vi "Compare Ports.vi"(9 "refresh listbox":T8[](array[typedef]), 10 "new port":T1, 11 "old port":T1) -> (1 "refresh listbox out":T8[](array[typedef]))   [LabVIEW 2020, in "Ballard ARINC 429 System Explorer.lvlib" / "Implementation.lvlib"]
uses:
  Implementation.lvlib
  Types/Refresh Listbox.ctl
  Types/Refresh Symbols.ctl
  Shared/VS Channels Definition for All Labels on Hardware Channel.ctl
  Shared/Direction.ctl
  Shared/VS Channels Definition for Label.ctl
  Shared/VS Channel Definition for Parameter.ctl
  Shared/Parameter Definition.ctl
  <vilib>/NI/NI VeriStand Encoding and Decoding/Encoding.ctl
  Shared/Transfer Type.ctl
  <vilib>/NI/NI VeriStand Encoding and Decoding/Encoding and Decoding.lvlib
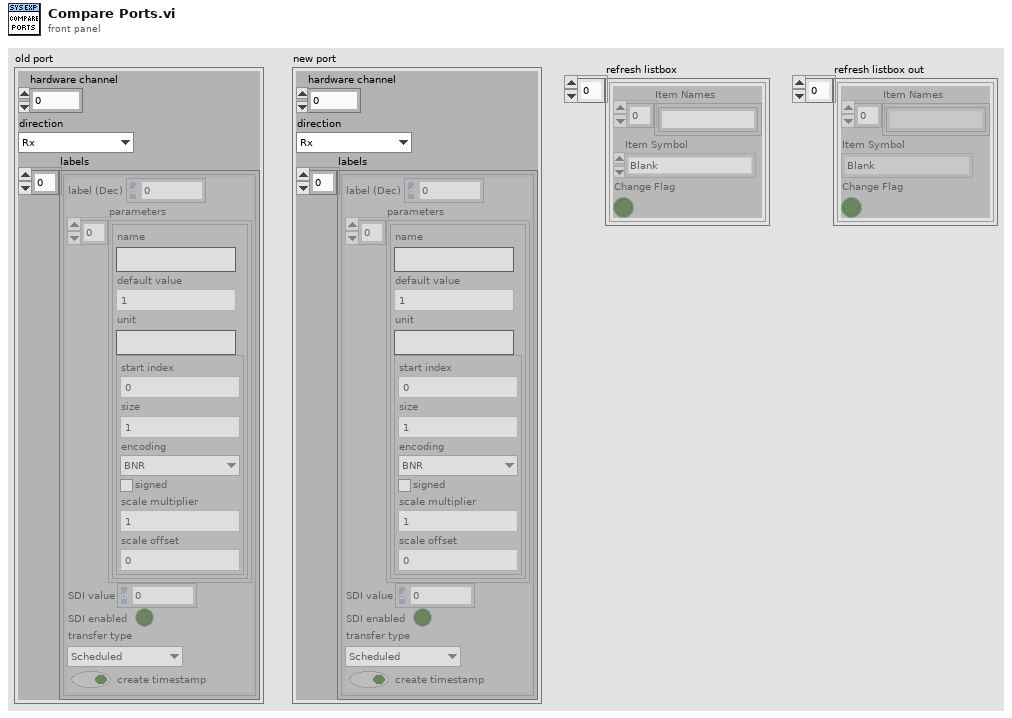
[diagram p1: front panel]
types:
  T1 = typedef "VS Channels Definition for All Labels on Hardware Channel.ctl" = cluster{"hardware channel":i32, "direction":T2, "labels":T3[]}
  T2 = typedef "Direction.ctl" = enum16{"Rx", "Tx"}
  T3 = typedef "VS Channels Definition for Label.ctl" = cluster{"label (Dec)":u32, "parameters":T4[], "SDI value":u8, "SDI enabled":bool, "transfer type":T7, "create timestamp":bool}
  T4 = typedef "VS Channel Definition for Parameter.ctl" = cluster{"name":string, "default value":dbl, "unit":string, "Parameter":T5}
  T5 = typedef "Parameter Definition.ctl" = cluster{"start index":i32, "size":i32, "encoding":T6, "signed":bool, "scale multiplier":dbl, "scale offset":dbl}
  T6 = typedef "Encoding and Decoding.lvlib/Encoding.ctl" = enum16{"BNR", "BCD", "Discrete"}
  T7 = typedef "Transfer Type.ctl" = enum16{"Scheduled", "Acyclic", "Block", "Strobe"}
  T8 = typedef "Ballard ARINC 429 System Explorer.lvlib/Implementation.lvlib/Refresh Listbox.ctl" = cluster{"Item Names":string[], "Item Symbol":T9, "Change Flag":bool}
  T9 = typedef "Ballard ARINC 429 System Explorer.lvlib/Implementation.lvlib/Refresh Symbols.ctl" = enum16{"Blank", "Port", "Incoming", "Outgoing", "Label", "Word", "Parameter", "ARINC-429", "Config Files", "Channel Spec", "Item"}
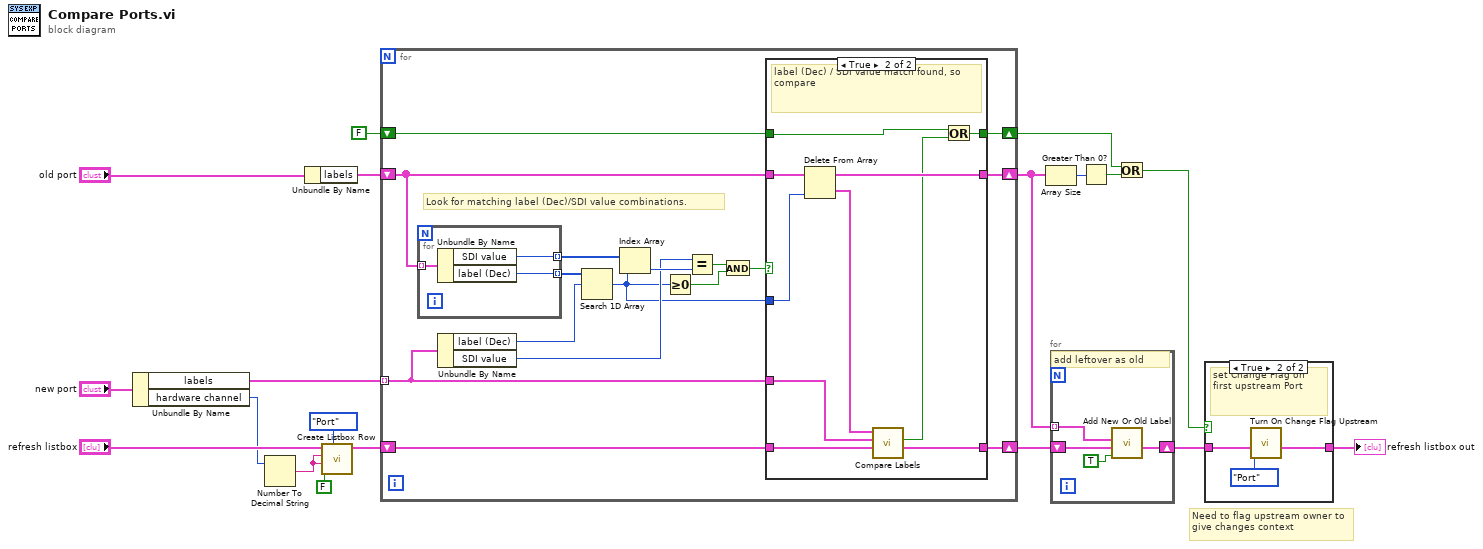
[diagram p0: block diagram]
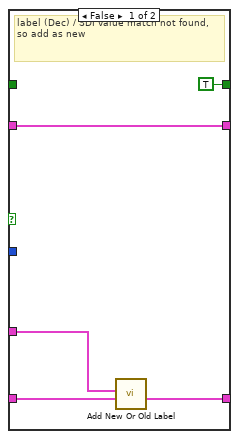
[diagram p3: hidden frame]
diagram:
  # "Need to flag upstream owner to give changes context"
  n1 = Unbundle By Name("new port") -> ("labels"=w16:T3[], "hardware channel"=w14:i32)
  n2 = Number To Decimal String(number=w14) -> (decimal integer string=w11:string)  [unwired: 1 in]
  n3 = Unbundle By Name("old port") -> ("labels"=w12:T3[])
  n4 = call "Create Listbox Row.vi"("refresh symbol (Blank)"=Refresh_Symbols."Port" ("Refresh Symbol (Blank)"), "change? (T)"=FALSE, "new item"=w11, "old item"=w11, "refresh listbox"="refresh listbox") -> ("refresh listbox out"=w15:T8[])  [unwired: 6 in]
  n5 = for {
    tunnel: w16 -> [w32] mode=indexing
    shift-right: [w34] -> w9
    shift-left: w15 -> [w35]
    shift-right: [w23] -> w5
    shift-left: w12 -> [w24]
    shift-right: [w20] -> w4
    shift-left: FALSE -> [w21]
    # "Look for matching label (Dec)/SDI value combinations."
    n6 = for {
      tunnel: w24 -> [w53] mode=indexing
      tunnel: [w52] -> w33 mode=indexing
      tunnel: [w51] -> w30 mode=indexing
      n7 = Unbundle By Name(w53) -> ("SDI value"=w51:u8, "label (Dec)"=w52:u32)
    }
    n8 = Unbundle By Name(w32) -> ("label (Dec)"=w31:u32, "SDI value"=w28:u8)
    n9 = Search 1D Array(1D array=w33, element=w31) -> (index of element=w22:i32)  [unwired: 1 in]
    n10 = Index Array(array=w30, index=w22) -> (element=w29:u8)
    n11 = Greater Or Equal To 0?(x=w22) -> (x >= 0?=w26:bool)
    n12 = Equal?(x=w28, y=w29) -> (x = y?=w27:bool)
    n13 = And(x=w27, y=w26) -> (x .and. y?=w25:bool)
    n14 = case shown="True" w25 {
      tunnel: w35 -> [w37 w46]
      tunnel: [w38 w47] -> w34
      tunnel: w32 -> [w39 w45]
      tunnel: w24 -> [w40 w50]
      tunnel: [w40 w48] -> w23
      tunnel: w22 -> [_ w49]
      tunnel: w21 -> [_ w41]
      tunnel: [TRUE w43] -> w20
      frame False {
        # "label (Dec) / SDI value match not found, so add as new"
        n15 = call "Add New Or Old Label.vi"("refresh listbox"=w37, "label"=w39) -> ("refresh listbox out"=w38:T8[])  [unwired: 9 in]
      }
      frame True {
        # "label (Dec) / SDI value match found, so compare"
        n16 = Delete From Array(array=w50, index=w49) -> (deleted portion=w44:T3, array with subset deleted=w48:T3[])  [unwired: 1 in]
        n17 = call "Compare Labels.vi"("refresh listbox"=w46, "new label"=w45, "old label"=w44) -> ("refresh listbox out"=w47:T8[], "any changes?"=w42:bool)  [unwired: 7 in]
        n18 = Or(x=w41, y=w42) -> (x .or. y?=w43:bool)
      }
    }
  }
  n19 = Array Size(array=w5) -> (size(s)=w6:i32)
  n20 = for {
    shift-right: [w56] -> w3
    shift-left: w9 -> [w57]
    tunnel: w5 -> [w55] mode=indexing
    # "add leftover as old"
    n21 = call "Add New Or Old Label.vi"("old label?"=TRUE, "refresh listbox"=w57, "label"=w55) -> ("refresh listbox out"=w56:T8[])  [unwired: 8 in]
  }
  n22 = Greater Than 0?(x=w6) -> (x > 0?=w7:bool)
  n23 = Or(x=w4, y=w7) -> (x .or. y?=w2:bool)
  n24 = case shown="True" w2 {
    tunnel: w3 -> [w58 w61]
    tunnel: [w58 w60] -> w1
    frame False {
    }
    frame True {
      # "set Change Flag on first upstream Port"
      n25 = call "Turn On Change Flag Upstream.vi"("symbol to change"=Refresh_Symbols."Port", "refresh listbox"=w61) -> ("refresh listbox out"=w60:T8[])  [unwired: 9 in]
    }
  }
  "refresh listbox out" <- w1
